vi "Parameters_Get_Stop.vi"(11 "Parameters":dbl[](array[numeric])) -> (3 "Stop Mode":i32(ring)=11599968 items=["Decelerate"=11599968, "Immediate"=11599969, "Disable Drive"=11599970])   [LabVIEW 2017, in "WordManipulationLibrary.lvlib"]
uses:
  WordManipulationLibrary.lvlib
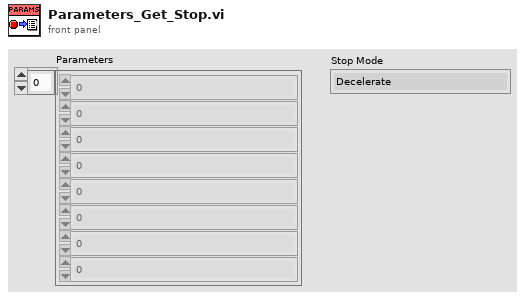
[diagram p1: front panel]
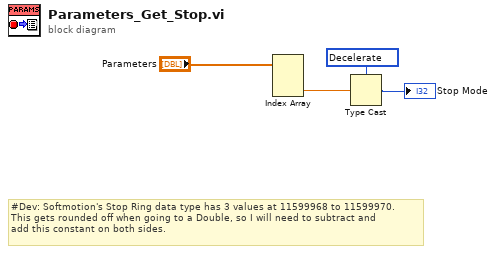
[diagram p0: block diagram]
diagram:
  w1 = 11599968 items=["Decelerate"=11599968, "Immediate"=11599969, "Disable Drive"=11599970] ("Stop Mode 2")
  # "#Dev: Softmotion's Stop Ring data type has 3 values at 11599968 to 11599970. \nThis gets rounded off when going to a Double, so I will need to subtract and\nadd this constant on both sides."
  n1 = Index Array(array="Parameters") -> (element #3=w3:dbl)  [unwired: 3 in, 2 out]
  n2 = Type Cast(type=w1, x=w3) -> (*(type *) &x=→"Stop Mode":i32)
